vi "CSE - Script Path & Search Paths.vi"(6 "action":enum32{"get", "save"}(ring), 8 "error in":errorcluster, 9 "search paths":path[](array[path]), 10 "script file path":path, 11 "CSE RefNum":T1) -> (0 "error out":errorcluster, 1 "search paths out":path[](array[path]), 2 "script file path out":path, 3 "dup CSE RefNum":T1)   [LabVIEW 2021]
doc: "This VI associates <b>script file path</b> and an array of <b>search paths</b> with the specified parsed script. CSE uses these paths if the script invokes another script using a relative file path. Refer to the VI help for more details.\n\n<b>CSE RefNum</b> must contain a reference to a CSE instance context containing a parsed script.\n\n<b>action</b> control specifies the operation to perform:\n 'get' : returns the paths associated with the script.\n 'save' : associates paths with the script.\n\n::: CalcExpress Toolkit :::\nCopyright (c) 2000-2026 Konstantin Shifershteyn. All rights reserved."
uses:
  CSE Instance RefNum.ctl
  cersrc/celveng32.dll
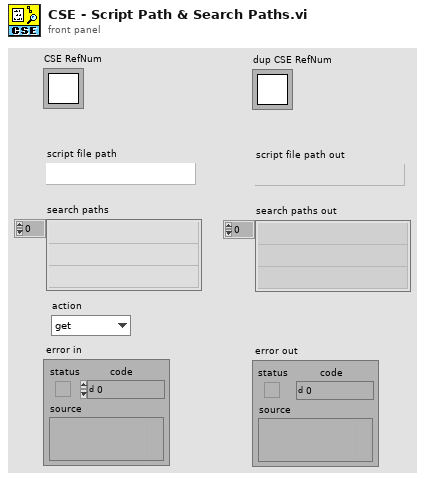
[diagram p1: front panel]
types:
  T1 = typedef "CSE Instance RefNum.ctl" = refnum<k1>
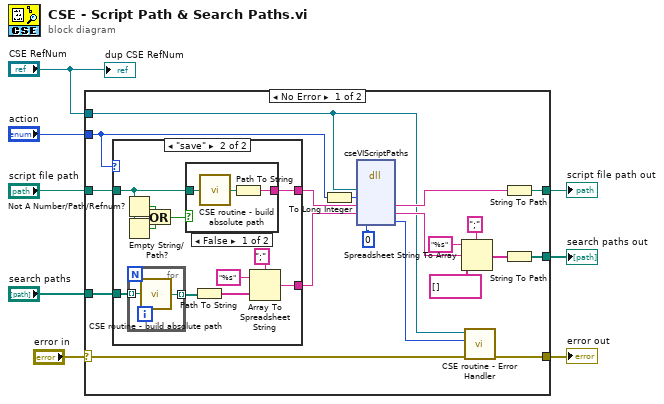
[diagram p0: block diagram]
diagram:
  n1 = case shown="No Error" "error in" {
    selector: "error in" -> [w11 w44]
    tunnel: "action" -> [w25 _]
    tunnel: "script file path" -> [w27 w46]
    tunnel: "search paths" -> [w26 w45]
    tunnel: "CSE RefNum" -> [w12 _]
    tunnel: [w21 w46] -> w4
    tunnel: [w14 w45] -> w3
    tunnel: [w10 w44] -> w1
    frame No Error {
      n2 = case shown="\"save\"" w25 {
        tunnel: [_ w35] -> w24
        tunnel: [_ w34] -> w23
        tunnel: w27 -> [_ w29]
        tunnel: w26 -> [_ w33]
        frame "get" {
        }
        frame "save" {
          n3 = Not A Number/Path/Refnum?(number/path/refnum=w29) -> (NaN/Path/Refnum?=w31:bool)
          n4 = Empty String/Path?(string/path=w29) -> (empty?=w30:bool)
          n5 = for {
            tunnel: w33 -> [w43] mode=indexing
            tunnel: [w42] -> w32 mode=indexing
            n6 = call "CSE routine - build absolute path.vi"("path in"=w43) -> ("path out"=w42:path)  [unwired: 4 in]
          }
          n7 = Or(x=w31, y=w30) -> (x .or. y?=w28:bool)
          n8 = case shown="False" w28 {
            tunnel: [w41 _] -> w35
            tunnel: w29 -> [w39 _]
            frame False {
              n9 = call "CSE routine - build absolute path.vi"("path in"=w39) -> ("path out"=w40:path)  [unwired: 4 in]
              n10 = Path To String(path=w40) -> (string=w41:string)
            }
            frame True {
            }
          }
          n11 = Path To String(path=w32) -> (string=w38:string[])
          n12 = Array To Spreadsheet String(delimiter (Tab)=";", array=w38, 3:"%s" ("format string")) -> (spreadsheet string=w34:string)
        }
      }
      n13 = To Long Integer(number=w25) -> (32bit integer=w9:i32)
      n14 = dll-call lib="C:/LV Projects/CalcExpress 40 LV2021/vi.lib/addons/CalcExpress/cersrc/celveng*.dll" fn="cseVIScriptPaths"("iRef"=w12, "cmd"=w9, "scrPath"=w24, "Paths"=w23, "erStat"=0) -> ("scrPath"=w20:string, "Paths"=w19:string, "erStat"=w13:i32)  [unwired: 6 in, 2 out]
      n15 = Spreadsheet String To Array(delimiter (Tab)=";", format string="%s", spreadsheet string=w19, array type (2D Dbl)=string[] []) -> (array=w15:string[])
      n16 = call "CSE routine - Error Handler.vi"("error in"=w11, "exec status"=w13, "CSE RefNum"=w12) -> ("error out"=w10:errorcluster)  [unwired: 4 in, 2 out]
      n17 = String To Path(string=w20) -> (path=w21:path)
      n18 = String To Path(string=w15) -> (path=w14:path[])
    }
    frame Error {
    }
  }
  "script file path out" <- w4
  "search paths out" <- w3
  "error out" <- w1
  "dup CSE RefNum" <- "CSE RefNum"
